vi "Build Unsupported Version Error.vi"(8 "error in":errorcluster, 11 "requested version":string) -> (0 "error out":errorcluster, 3 "payload":string)   [LabVIEW 2020, in "MCP Server.lvlib"]
doc: "Builds the JSON-RPC error for an unsupported protocol version, in the form MCP 2026-07-28 defines so that dual-era clients recognise a modern server: {\"jsonrpc\":\"2.0\",\"id\":null,\"error\":{\"code\":-32022,\"message\":\"Unsupported protocol version\",\"data\":{\"supported\":[all versions],\"requested\":\"<version>\"}}}. supported lists all versions of Supported Protocol Versions.vi, modern and legacy. Answered with HTTP 400, in both eras."
uses:
  MCP Server.lvlib
  9d621cb8-1402-48c2-83a0-11e0b8cd24b7.vi
  1b7ccd26-b579-4bf5-9d29-0438f1ba35eb.vi
  <vilib>/JDP Science/JSONtext/Variant to JSON Text.vi
  <vilib>/JDP Science/JSONtext/LVClass Serializer/JSONtext LVClass Serializer.lvclass
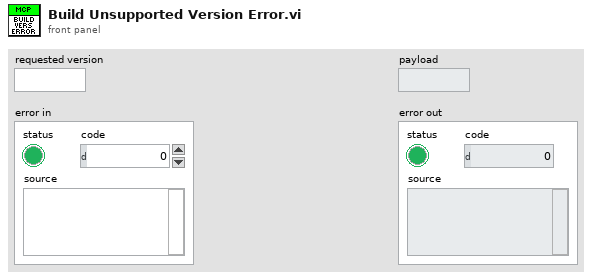
[diagram p1: front panel]
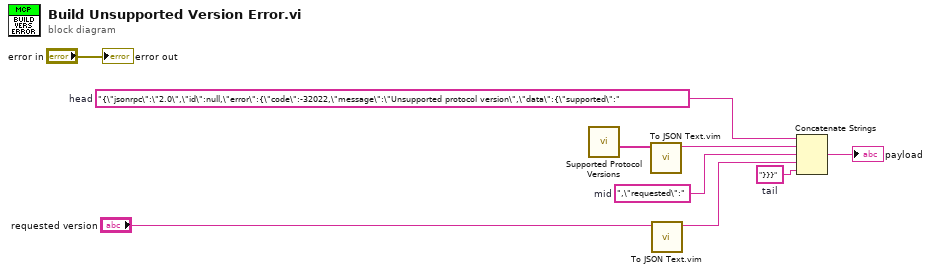
[diagram p0: block diagram]
diagram:
  w3 = "}}}"  # tail
  w5 = ",\"requested\":"  # mid
  w7 = "{\"jsonrpc\":\"2.0\",\"id\":null,\"error\":{\"code\":-32022,\"message\":\"Unsupported protocol version\",\"data\":{\"supported\":"  # head
  n1 = call "Supported Protocol Versions.vi"() -> ("all versions"=w9:string[])  [unwired: 9 in, 2 out]
  n2 = call "To JSON Text.vim"("Anything"=w9) -> ("<JSON>"=w6:string)  [unwired: 9 in, 1 out]
  n3 = call "To JSON Text.vim"("Anything"="requested version") -> ("<JSON>"=w4:string)  [unwired: 9 in, 1 out]
  n4 = Concatenate Strings(w7, w6, w5, w4, w3) -> (→"payload":string)
  "error out" <- "error in"
